vi "meas_osc_2021.vi"() -> ()   [LabVIEW 2019]
uses:
  <instrlib>/Agilent 2000 3000 X-Series/Public/Configure/Configure Timebase (Basic).vi
  <instrlib>/Agilent 2000 3000 X-Series/Public/Data/Read Measurement (Current Value).vi
  <instrlib>/Agilent 2000 3000 X-Series/Agilent 2000 3000 X-Series.lvlib
panel:
  in  "Scale (50 s/div)":dbl=50.0
  in  "Coupling (1: DC)":i32(ring)=1 items=["AC", "DC"]
  in  "Vertical Scale (5.0 V)":dbl=5.0
  in  "Channel Name (0: Channel 1)":i32(ring) items=["Channel 1", "Channel 2", "Channel 3", "Channel 4"]
  in  "Measurement Type (0: Peak-Peak)":i32(ring) items=["Peak-Peak", "Maximum", "Minimum", "Amplitude", "Top", "Base", "Overshoot", "Preshoot", "Average - N Cycles", "Average - Full Screen", "DC RMS - N Cycles", "DC RMS - Full Screen", "AC RMS - N Cycles", "AC RMS - Full Screen (Std Dev)", "Ratio", "Period", "Frequency", "Counter", "+Width", "-Width", "Burst Width", "Duty Cycle", "Rise Time", "Fall Time", "Delay", "Phase", "X minY", "X maxY", "Positive Pulse Count", "Negative Pulse Count", "Raising Edge Count", "Falling Edge Count", "Area - N Cycle", "Area - Full Screen", "Nth Edge Time", "Nth Edge Cross Level Time"]
  out "Result Value":dbl
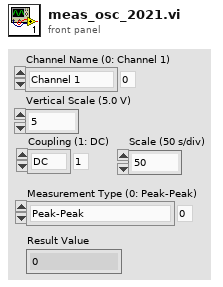
[diagram p1: front panel]
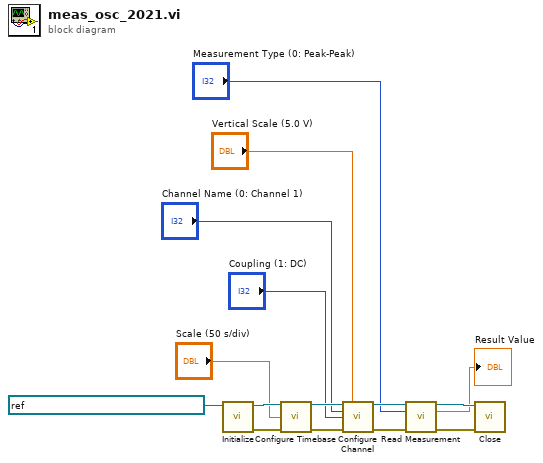
[diagram p0: block diagram]
diagram:
  n1 = call <instrlib>:"Initialize.vi"("VISA resource name"=refnum<visa-resource-name> "TCPIP0::192.168.2.2::inst0::INSTR") -> ("error out"=w3:errorcluster, "VISA resource name out"=w4:refnum<visa-resource-name>)  [unwired: 9 in]
  n2 = call-poly <instrlib>:"Configure Timebase.vi"("VISA resource name"=w4, "Scale (50 s/div)"="Scale (50 s/div)", "error in (no error)"=w3) -> ("VISA resource name out"=w15:refnum<visa-resource-name>, "error out"=w14:errorcluster)  [unwired: 11 in]
  n3 = call <instrlib>:"Configure Channel.vi"("VISA resource name"=w15, "Vertical Scale (5.0 V)"="Vertical Scale (5.0 V)", "Channel Name (0: Channel 1)"="Channel Name (0: Channel 1)", "Coupling (1: DC)"="Coupling (1: DC)", "error in (no error)"=w14) -> ("VISA resource name out"=w13:refnum<visa-resource-name>, "error out"=w12:errorcluster)  [unwired: 9 in]
  n4 = call-poly <instrlib>:"Read Measurement.vi"("VISA resource name"=w13, "Measurement Type (0: Peak-Peak)"="Measurement Type (0: Peak-Peak)", "error in (no error)"=w12) -> ("VISA resource name out"=w10:refnum<visa-resource-name>, "Result Value"=→"Result Value":dbl, "error out"=w11:errorcluster)  [unwired: 10 in]
  n5 = call <instrlib>:"Close.vi"("error in (no error)"=w11, "VISA resource name"=w10) -> ()  [unwired: 9 in, 1 out]
